vi "Abort Stream.vi"(8 "error in (no error)":errorcluster, 11 "MCP SSE Response in":refnum<class "MCP SSE Response.lvclass">) -> (0 "error out":errorcluster, 3 "MCP SSE Response out":refnum<class "MCP SSE Response.lvclass">)   [LabVIEW 2020, in "MCP Server.lvlib" / "MCP SSE Response.lvclass"]
doc: "Called by the IG HTTP Server when the stream is abandoned. Sets the cancelled flag (a single-element queue) to TRUE so that code producing the events can see that the client is gone. The queues are not released here; their creator owns them."
uses:
  MCP SSE Response.lvclass
  MCP SSE Response.lvclass/MCP SSE Response.ctl
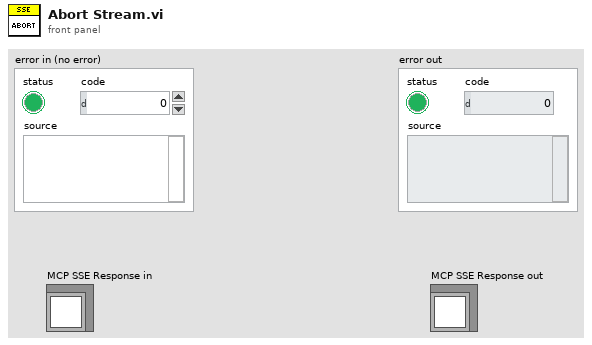
[diagram p1: front panel]
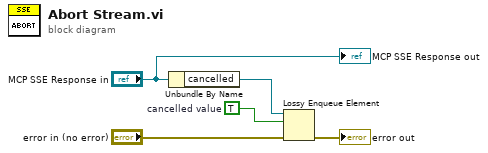
[diagram p0: block diagram]
diagram:
  w4 = TRUE  # cancelled value
  n1 = Unbundle By Name("MCP SSE Response in") -> ("cancelled"=w5:refnum<queue>)
  n2 = Lossy Enqueue Element(queue=w5, element=w4, error in (no error)="error in (no error)") -> (error out=→"error out":errorcluster)  [unwired: 3 out]
  "MCP SSE Response out" <- "MCP SSE Response in"
